vi "PromVIEW Basic Metrics Example.vi"() -> ()   [LabVIEW 2020]
uses:
  src/metrics/gauge/Gauge.lvclass
  src/metrics/counter/Counter.lvclass
  src/registry/session/Registry Session.lvclass
panel:
  in  "Area 2":picture
  in  "Area 1":picture
  # "Instructions: \n- See the Readme.md file from the project to see how to expose metrics collected by this VI.\n- Run this VI.\n- Start clicking in areas above. Metrics collecting the number of clicks will be exposed by the PromTest1 webservice"
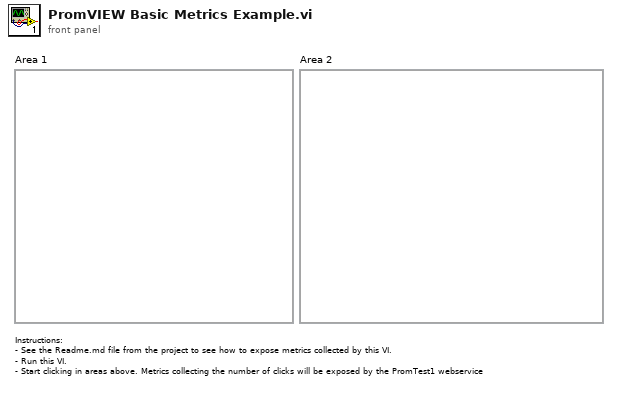
[diagram p1: front panel]
types:
  T1 = typedef "Registry.lvlib/Registry Session.lvclass/Session Handle.ctl" = refnum<data-value>
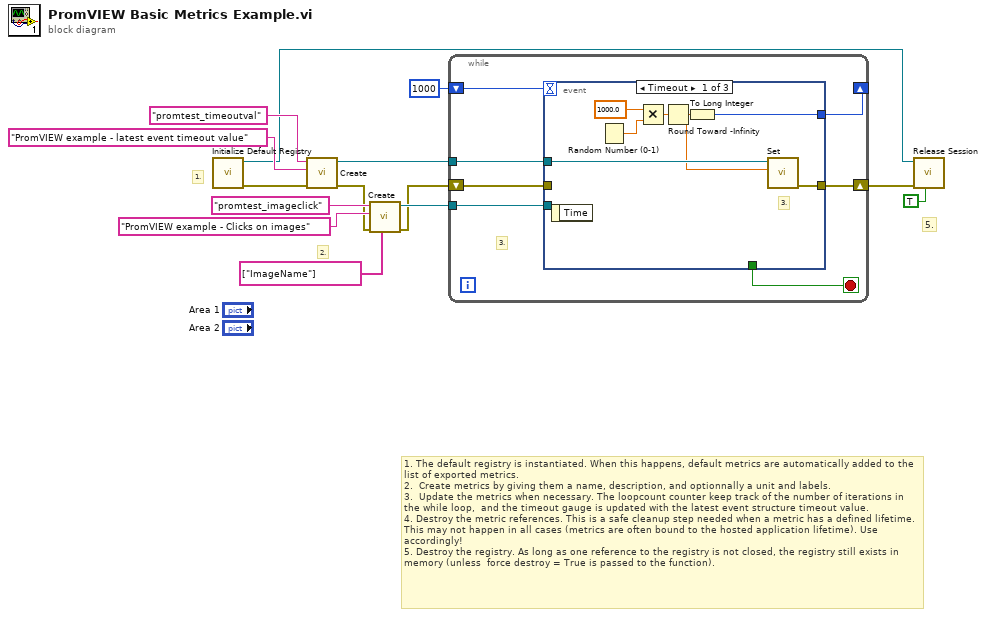
[diagram p0: block diagram]
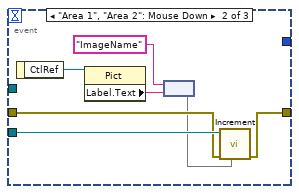
[diagram p2: hidden frame]
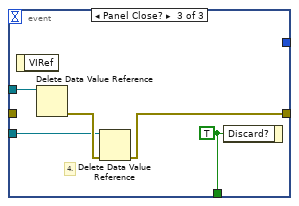
[diagram p3: hidden frame]
diagram:
  # "1. The default registry is instantiated. When this happens, default metrics are automatically added to the list of exported metrics.\n2.  Create metrics by giving them a name, description, and optionnally a unit and labels.\n3.  Update the metrics when necessary. The loopcount counter keep track of the number of iterations in the while loop,  and the timeout gauge is updated with the latest event structure timeout value.\n4. Destroy the metric references. This is a safe cleanup step needed when a metric has a defined lifetime. This may not happen in all cases (metrics are often bound to the hosted application lifetime). Use accordingly!\n5. Destroy the registry. As long as one reference to the registry is not closed, the registry still exists in memory (unless  force destroy = True is passed to the function)."
  # "5."
  # "2."
  # "1."
  n1 = call "Initialize Default Registry.vi"() -> ("error out"=w13:errorcluster, "Session Handle"=w6:T1)  [unwired: 9 in, 1 out]
  n2 = call "Create.vi"("error in (no error)"=w13, "Description"="PromVIEW example - latest event timeout value", "Metric Name"="promtest_timeoutval") -> ("error out"=w3:errorcluster, "Gauge Ref"=w8:refnum<data-value>)  [unwired: 7 in]
  n3 = call "Create.vi"("Label Names"=string[] ["ImageName"], "error in (no error)"=w3, "Description"="PromVIEW example - Clicks on images", "Metric Name"="promtest_imageclick") -> ("error out"=w2:errorcluster, "Counter Ref"=w7:refnum<data-value>)  [unwired: 6 in]
  n4 = while {
    shift-right: [w20] -> _
    shift-left: 1000 -> [w19]
    tunnel: w8 -> [w18]
    tunnel: w7 -> [w16]
    shift-right: [w17] -> w5
    shift-left: w2 -> [w15]
    stop <- w21 stop-if-true
    # "3."
    n5 = event shown="[0] Timeout" {
      selector: _ -> [_ _ _]
      dyn-events: _ -> [_ _ _]
      timeout: w19 -> [_ _ _]
      tunnel: [_ _ w40] -> w21
      tunnel: [w23 _ _] -> w20
      tunnel: w18 -> [w25 _ w39]
      tunnel: [w22 w32 w37] -> w17
      tunnel: w16 -> [_ w34 w36]
      tunnel: w15 -> [_ w33 _]
      event Timeout {
        # "3."
        n6 = event-data() -> ()  [unwired: 1 in, 1 out]
        n7 = Random Number (0-1)() -> (number: 0 to 1=w28:dbl)
        n8 = Multiply(x=1000.0, y=w28) -> (x*y=w26:dbl)
        n9 = Round Toward -Infinity(1:w26) -> (0:w24:dbl)
        n10 = To Long Integer(number=w24) -> (32bit integer=w23:i32)
        n11 = call "Set.vi"("Value"=w24, "Gauge Ref"=w25) -> ("error out"=w22:errorcluster)  [unwired: 8 in, 1 out]
      }
      event "Area 1", "Area 2": Mouse Down {
        n12 = event-data() -> ("CtlRef"=w35:refnum<vi>)  [unwired: 1 in]
        n13 = property class="Pict"(reference=w35) -> ("Label.Text"=w30:string)  [unwired: 1 in, 2 out]
        n14 = node("ImageName" ("Labelname"), w30) -> (w29:map{string, string})
        n15 = call "Increment.vi"("Labels"=w29, "error in (no error)"=w33, "Counter Ref"=w34) -> ("error out"=w32:errorcluster)  [unwired: 7 in, 1 out]
      }
      event Panel Close? {
        w40 = TRUE ("Discard?")
        # "4."
        n16 = event-data() -> ()  [unwired: 1 in, 1 out]
        n17 = Delete Data Value Reference(data value reference=w39) -> (error out=w38:errorcluster)  [unwired: 1 in, 1 out]
        n18 = Delete Data Value Reference(data value reference=w36, error in=w38) -> (error out=w37:errorcluster)  [unwired: 1 out]
        n19 = event-data("Discard?"=w40) -> ()  [unwired: 1 in, 1 out]
      }
    }
  }
  n20 = call "Release Session.vi"("force destroy? (F)"=TRUE, "error in (no error)"=w5, "Session Handle"=w6) -> ()  [unwired: 8 in, 1 out]
